vi "Step_Editor.vi"(8 "error in (no error)":errorcluster={"status"=FALSE, "code"=0, "source"="\"\""}, 10 "parameter registry":string, 11 "ActionDefinition":string) -> (0 "error out":errorcluster={"status"=FALSE, "code"=0, "source"="\"\""}, 2 "status ok":bool, 3 "Updated action":string)   [LabVIEW 2026]
doc: "INTENT: Edit action parameters. LOGIC: Select action type, commands, deadlines, feedback/timeout/retry/capture configuration; validate units."
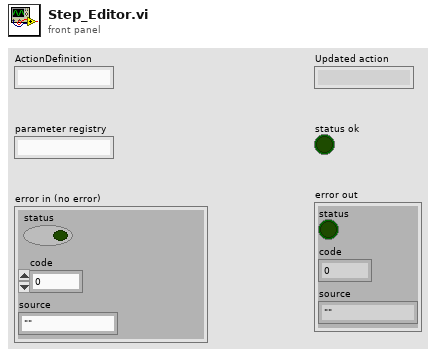
[diagram p1: front panel]
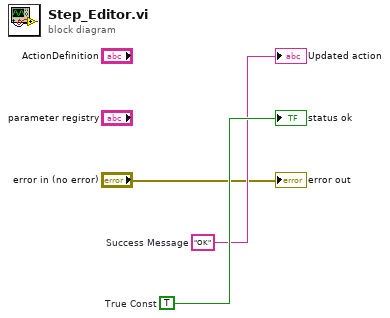
[diagram p0: block diagram]
diagram:
  w3 = TRUE  # True Const
  w2 = "OK"  # Success Message
  "Updated action" <- w2
  "status ok" <- w3
  "error out" <- "error in (no error)"
